vi "cam_dinamic_roi_set_3.vi"(4 "Right_center":dbl, 6 "Right Descriptor":T1 {"Contours"."Type" items=["No Selection", "Point", "Line", "Rectangle", "Oval", "Polygon", "Freehand Region", "Annulus", "Unused2", "Unused3", "Broken Line", "Freehand Line", "Rotated Rectangle"]}, 7 "Lane Descriptor":T1 {"Contours"."Type" items=["No Selection", "Point", "Line", "Rectangle", "Oval", "Polygon", "Freehand Region", "Annulus", "Unused2", "Unused3", "Broken Line", "Freehand Line", "Rotated Rectangle"]}, 8 "steer(deg)":dbl, 9 "Left_center":dbl, 10 "Left Descriptor":T1 {"Contours"."Type" items=["No Selection", "Point", "Line", "Rectangle", "Oval", "Polygon", "Freehand Region", "Annulus", "Unused2", "Unused3", "Broken Line", "Freehand Line", "Rotated Rectangle"]}, 11 "Lane_center":dbl) -> (1 "Right":T2, 2 "Left":T2, 3 "Mid":T2)   [LabVIEW 2024]
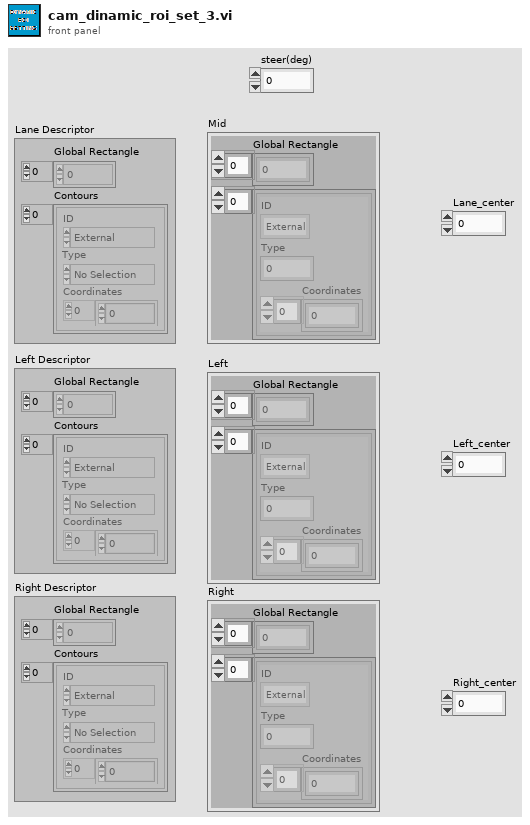
[diagram p1: front panel]
types:
  T1 = typedef "ROI Descriptor" = cluster{"Global Rectangle":i32[], "Contours":cluster{"ID":enum32{"External", "Internal"}, "Type":u32, "Coordinates":i32[]}[]}
  T2 = cluster{"Global Rectangle":i32[], cluster{"ID":enum32{"External", "Internal"}, "Type":u32, "Coordinates":i32[]}[]}
  T3 = cluster{"ID":enum32{"External", "Internal"}, "Type":u32, "Coordinates":i32[]}[]
  T4 = cluster{"ID":enum32{"External", "Internal"}, "Type":u32, "Coordinates":i32[]}
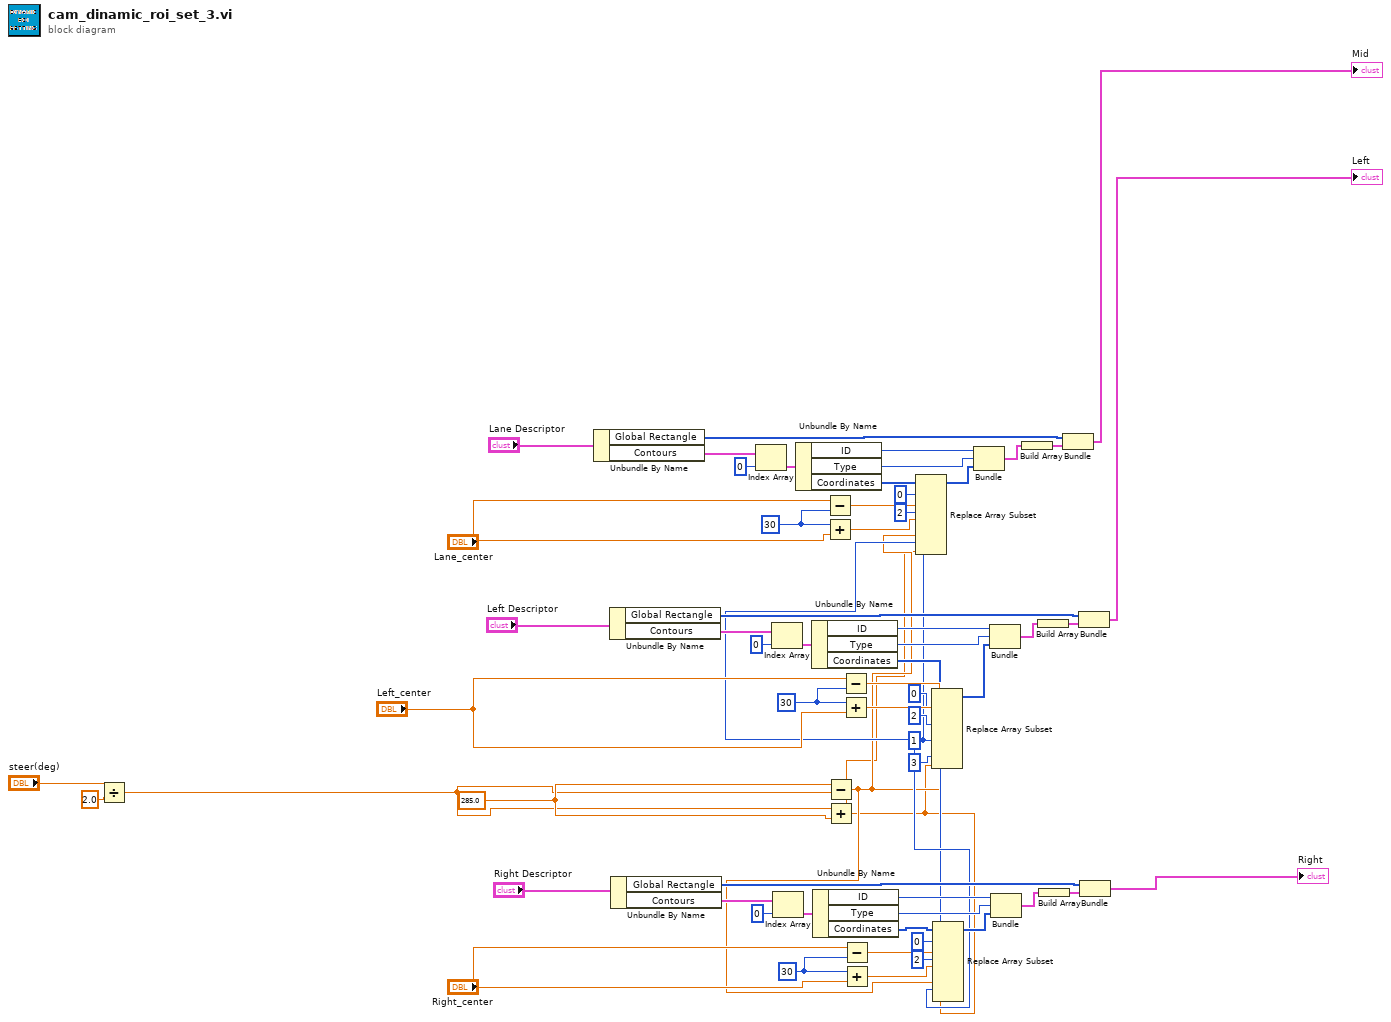
[diagram p0: block diagram]
diagram:
  w6 = 285.0 ("x")
  w8 = 3 ("index")
  w7 = 1 ("index")
  w43 = 30
  w38 = 30
  w11 = 30
  n1 = Divide(x="steer(deg)", y=2.0) -> (x/y=w1:dbl)
  n2 = Unbundle By Name("Lane Descriptor") -> ("Global Rectangle"=w17:i32[], "Contours"=w23:T3)
  n3 = Unbundle By Name("Left Descriptor") -> ("Global Rectangle"=w32:i32[], "Contours"=w26:T3)
  n4 = Unbundle By Name("Right Descriptor") -> ("Global Rectangle"=w49:i32[], "Contours"=w55:T3)
  n5 = Index Array(array=w23, index=0 ("인덱스")) -> (element=w22:T4)
  n6 = Index Array(array=w26, index=0 ("인덱스")) -> (element=w27:T4)
  n7 = Index Array(array=w55, index=0 ("인덱스")) -> (element=w54:T4)
  n8 = Unbundle By Name(w22) -> ("ID"=w16:enum32{"External", "Internal"}, "Type"=w15:u32, "Coordinates"=w18:i32[])
  n9 = Unbundle By Name(w27) -> ("ID"=w33:enum32{"External", "Internal"}, "Type"=w34:u32, "Coordinates"=w31:i32[])
  n10 = Unbundle By Name(w54) -> ("ID"=w48:enum32{"External", "Internal"}, "Type"=w47:u32, "Coordinates"=w50:i32[])
  n11 = Subtract(x="Lane_center", y=w11) -> (x-y=w10:dbl)
  n12 = Add(x=w11, y="Lane_center") -> (x+y=w9:dbl)
  n13 = Subtract(x=w6, y=w1) -> (x-y=w5:dbl)
  n14 = Add(x=w1, y=w6) -> (x+y=w4:dbl)
  n15 = Subtract(x="Left_center", y=w38) -> (x-y=w39:dbl)
  n16 = Add(x=w38, y="Left_center") -> (x+y=w40:dbl)
  n17 = Subtract(x="Right_center", y=w43) -> (x-y=w42:dbl)
  n18 = Add(x=w43, y="Right_center") -> (x+y=w41:dbl)
  n19 = Replace Array Subset(array=w18, new element #1=w10, index #1=0 ("인덱스"), new element #2=w9, index #2=2 ("인덱스"), new element #3=w5, index #3=w7, new element #4=w4, index #4=w8) -> (w14:i32[])
  n20 = Replace Array Subset(array=w31, new element #1=w39, index #1=0 ("인덱스"), new element #2=w40, index #2=2 ("인덱스"), new element #3=w5, index #3=w7, new element #4=w4, index #4=w8) -> (w35:i32[])
  n21 = Replace Array Subset(array=w50, new element #1=w42, index #1=0 ("인덱스"), new element #2=w41, index #2=2 ("인덱스"), new element #3=w5, index #3=w7, new element #4=w4, index #4=w8) -> (w46:i32[])
  n22 = Bundle("ID"=w16, "Type"=w15, "Coordinates"=w14) -> (w12:T4)  [unwired: 1 in]
  n23 = Bundle("ID"=w33, "Type"=w34, "Coordinates"=w35) -> (w37:T4)  [unwired: 1 in]
  n24 = Bundle("ID"=w48, "Type"=w47, "Coordinates"=w46) -> (w44:T4)  [unwired: 1 in]
  n25 = Build Array(w12) -> (w13:T3)
  n26 = Build Array(w37) -> (w36:T3)
  n27 = Build Array(w44) -> (w45:T3)
  n28 = Bundle("Global Rectangle"=w17, w13) -> (→"Mid":T2)  [unwired: 1 in]
  n29 = Bundle("Global Rectangle"=w32, w36) -> (→"Left":T2)  [unwired: 1 in]
  n30 = Bundle("Global Rectangle"=w49, w45) -> (→"Right":T2)  [unwired: 1 in]
